vi "ZMQ Rep Test.vi"() -> ()   [LabVIEW 2019, in "RemoteControl.ZMQ.lvlib" / "RemoteControl.ZMQ.lvclass"]
uses:
  RemoteControl.ZMQ.lvclass
  <userlib>/LevyLab/RemoteControl/RemoteControl/Typedefs/Message--Cluster.ctl
  C:/Program Files/National Instruments/LabVIEW 2019/user.lib/LevyLab/RemoteControl/RemoteControl/RemoteControl.lvclass
  <userlib>/LevyLab/RemoteControl/RemoteControl/RemoteControl.lvclass/RemoteControl.ctl
  <vilib>/addons/zeromq/zmq_context.lvclass
  <vilib>/addons/zeromq/socket_type.ctl
  <vilib>/addons/zeromq/zeromq.lvlib
  <vilib>/addons/zeromq/zmq_socket.lvclass
  <vilib>/addons/zeromq/socket_options.ctl
  <userlib>/LevyLab/RemoteControl/RemoteControl/RemoteControl.lvclass
panel:
  out "Message":T1
  out "error out":errorcluster
  in  "stop":bool
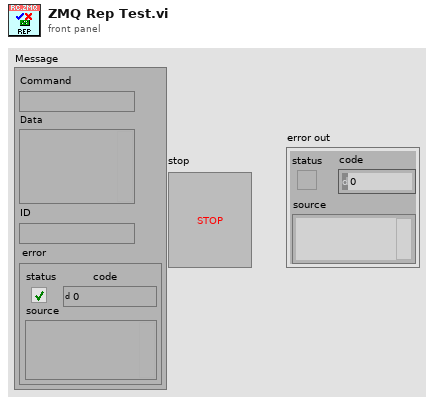
[diagram p1: front panel]
types:
  T1 = typedef "RemoteControl.lvlib/RemoteControl.lvclass/Message--Cluster.ctl" = cluster{"Command":string, "Data":variant, "ID":string, "error":errorcluster}
  T2 = typedef "zeromq.lvlib/socket_options.ctl" = enum8{"NONE", "ZMQ_HWM", "<2>", "ZMQ_SWAP", "ZMQ_AFFINITY", "ZMQ_ROUTING_ID", "ZMQ_SUBSCRIBE", "ZMQ_UNSUBSCRIBE", "ZMQ_RATE", "ZMQ_RECOVERY_IVL", "ZMQ_MCAST_LOOP", "ZMQ_SNDBUF", "ZMQ_RCVBUF", "ZMQ_RCVMORE", "ZMQ_FD", "ZMQ_EVENTS", "ZMQ_TYPE", "ZMQ_LINGER", "ZMQ_RECONNECT_IVL", "ZMQ_BACKLOG", "ZMQ_RECOVERY_IVL_MSEC", "ZMQ_RECONNECT_IVL_MAX", "ZMQ_MAXMSGSIZE", "ZMQ_SNDHWM", "ZMQ_RCVHWM", "ZMQ_MULTICAST_HOPS", "<26>", "ZMQ_RCVTIMEO", "ZMQ_SNDTIMEO", "<29>", "<30>", "ZMQ_IPV4ONLY", "ZMQ_LAST_ENDPOINT", "ZMQ_ROUTER_MANDATORY", "ZMQ_TCP_KEEPALIVE", "ZMQ_TCP_KEEPALIVE_CNT", "ZMQ_TCP_KEEPALIVE_IDLE", "ZMQ_TCP_KEEPALIVE_INTVL", "ZMQ_TCP_ACCEPT_FILTER", "ZMQ_IMMEDIATE", "ZMQ_XPUB_VERBOSE", "ZMQ_ROUTER_RAW", "ZMQ_IPV6", "ZMQ_MECHANISM", "ZMQ_PLAIN_SERVER", "ZMQ_PLAIN_USERNAME", "ZMQ_PLAIN_PASSWORD", "ZMQ_CURVE_SERVER", "ZMQ_CURVE_PUBLICKEY", "ZMQ_CURVE_SECRETKEY", "ZMQ_CURVE_SERVERKEY", "ZMQ_PROBE_ROUTER", "ZMQ_REQ_CORRELATE", "ZMQ_REQ_RELAXED", "ZMQ_CONFLATE", "ZMQ_ZAP_DOMAIN", "ZMQ_ROUTER_HANDOVER", "ZMQ_TOS", "ZMQ_IPC_FILTER_PID", "ZMQ_IPC_FILTER_UID", "ZMQ_IPC_FILTER_GID", "ZMQ_CONNECT_ROUTING_ID", "ZMQ_GSSAPI_SERVER", "ZMQ_GSSAPI_PRINCIPAL", "ZMQ_GSSAPI_SERVICE_PRINCIPAL", "ZMQ_GSSAPI_PLAINTEXT", "ZMQ_HANDSHAKE_IVL", "<67>", "ZMQ_SOCKS_PROXY", "ZMQ_XPUB_NODROP", "ZMQ_BLOCKY", "ZMQ_XPUB_MANUAL", "ZMQ_XPUB_WELCOME_MSG", "ZMQ_STREAM_NOTIFY", "ZMQ_INVERT_MATCHING", "ZMQ_HEARTBEAT_IVL", "ZMQ_HEARTBEAT_TTL", "ZMQ_HEARTBEAT_TIMEOUT", "ZMQ_XPUB_VERBOSER", "ZMQ_CONNECT_TIMEOUT", "ZMQ_TCP_MAXRT", "ZMQ_THREAD_SAFE", "<82>", "<83>", "ZMQ_MULTICAST_MAXTPDU", "ZMQ_VMCI_BUFFER_SIZE", "ZMQ_VMCI_BUFFER_MIN_SIZE", "ZMQ_VMCI_BUFFER_MAX_SIZE", "ZMQ_VMCI_CONNECT_TIMEOUT", "ZMQ_USE_FD", "ZMQ_GSSAPI_PRINCIPAL_NAMETYPE", "ZMQ_GSSAPI_SERVICE_PRINCIPAL_NAMETYPE", "ZMQ_BINDTODEVICE", "ZMQ_ZAP_ENFORCE_DOMAIN", "ZMQ_LOOPBACK_FASTPATH", "ZMQ_METADATA", "ZMQ_MULTICAST_LOOP", "ZMQ_ROUTER_NOTIFY"}
  T3 = typedef "zeromq.lvlib/socket_type.ctl" = enum8{"ZMQ_PAIR", "ZMQ_PUB", "ZMQ_SUB", "ZMQ_REQ", "ZMQ_REP", "ZMQ_DEALER", "ZMQ_ROUTER", "ZMQ_PULL", "ZMQ_PUSH", "ZMQ_XPUB", "ZMQ_XSUB", "ZMQ_STREAM", "ZMQ_SERVER", "ZMQ_CLIENT", "ZMQ_RADIO", "ZMQ_DISH", "ZMQ_GATHER", "ZMQ_SCATTER", "ZMQ_DGRAM"}
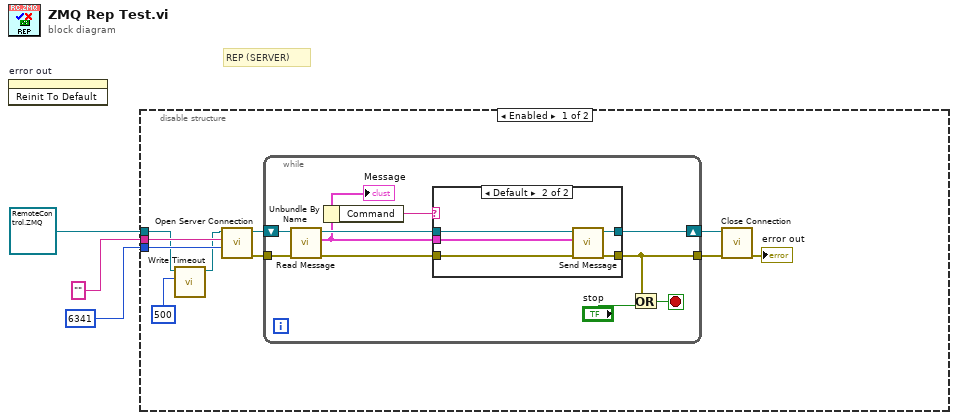
[diagram p0: block diagram]
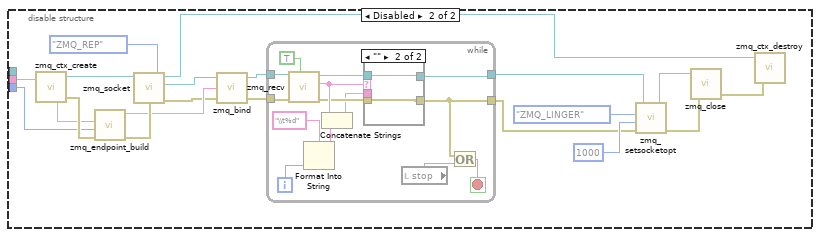
[diagram p3: hidden frame]
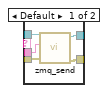
[diagram p4: hidden frame]
diagram:
  # "REP (SERVER)"
  n1 = invoke on="error out" class="Clust (strict)" method="Reinit To Default"() -> ()  [unwired: 3 in, 3 out]
  n2 = disable-structure shown="Enabled" {
    disable-tunnel: refnum<class "RemoteControl.ZMQ.lvclass"> refnum ("RemoteControl.ZMQ.lvlib:RemoteControl.ZMQ.lvclass") -> [w6 _]
    disable-tunnel: u16 6341 ("Port") -> [w9 w38]
    disable-tunnel: "" ("Address") -> [w8 w37]
    frame Enabled {
      n3 = call <userlib>:"Write Timeout.vi"("timeout (ms) [500]"=500 ("timeout in ms (100)"), "RemoteControl in"=w6) -> ("RemoteControl out"=w5:refnum<class "RemoteControl.ZMQ.lvclass">)  [unwired: 8 in, 1 out]
      n4 = call-dynamic "Open Server Connection.vi"("port"=w9, "address"=w8, "RemoteControl.ZMQ in"=w5) -> ("error out"=w12:errorcluster, "RemoteControl.ZMQ out"=w13:refnum<class "RemoteControl.ZMQ.lvclass">)  [unwired: 7 in]
      n5 = while {
        tunnel: w12 -> [w22]
        tunnel: [w18] -> w10
        shift-right: [w19] -> w11
        shift-left: w13 -> [w23]
        stop <- w17 stop-if-true
        n6 = call-dynamic "Read Message.vi"("error in (no error)"=w22, "RemoteControl.ZMQ in"=w23) -> ("error out"=w21:errorcluster, "Message"=w14:T1, "RemoteControl.ZMQ out"=w20:refnum<class "RemoteControl.ZMQ.lvclass">)  [unwired: 7 in]
        "Message" <- w14
        n7 = Unbundle By Name(w14) -> ("Command"=w15:string)
        n8 = case shown="Default" w15 {
          tunnel: w21 -> [w24 w30]
          tunnel: w20 -> [w25 w29]
          tunnel: [w25 w28] -> w19
          tunnel: [w24 w27] -> w18
          tunnel: w14 -> [_ w26]
          frame "" {
            # "no incoming msg:\ndo nothing"
          }
          frame Default {
            n9 = call-dynamic "Send Message.vi"("error in (no error)"=w30, "Message"=w26, "RemoteControl.ZMQ in"=w29) -> ("error out"=w27:errorcluster, "RemoteControl.ZMQ out"=w28:refnum<class "RemoteControl.ZMQ.lvclass">)  [unwired: 7 in]
          }
        }
        n10 = Or(x=w18, y="stop") -> (x .or. y?=w17:bool)
      }
      n11 = call-dynamic "Close Connection.vi"("error in (no error)"=w10, "RemoteControl.ZMQ in"=w11) -> ("error out"=→"error out":errorcluster)  [unwired: 8 in, 1 out]
    }
    frame Disabled {
      n12 = call <vilib>:"zmq_ctx_create.vi"() -> ("error out"=w47:errorcluster, "context out"=w49:refnum<class "zmq_context.lvclass">)  [unwired: 4 in]
      n13 = call <vilib>:"zmq_endpoint_build.vi"("error in"=w47, "port"=w38, "address"=w37) -> ("error out"=w46:errorcluster, "endpoint"=w35:string)  [unwired: 2 in, 1 out]
      n14 = call <vilib>:"zmq_socket.vi"("error in"=w46, "socket type"=socket_type."ZMQ_REP", "context in"=w49) -> ("error out"=w34:errorcluster, "socket out"=w36:refnum<class "zmq_socket.lvclass">, "context out"=w39:refnum<class "zmq_context.lvclass">)  [unwired: 2 in]
      n15 = call <vilib>:"zmq_bind.vi"("error in"=w34, "endpoint"=w35, "socket in"=w36) -> ("error out"=w32:errorcluster, "socket out"=w33:refnum<class "zmq_socket.lvclass">)  [unwired: 1 in]
      n16 = while {
        tunnel: w32 -> [w60]
        tunnel: w33 -> [w61]
        tunnel: [w58] -> w42
        tunnel: [w53] -> w31
        i -> [w56]
        stop <- w62 stop-if-true
        n17 = call <vilib>:"zmq_recv.vi"("no block? (F)"=TRUE, "error in"=w60, "socket in"=w61) -> ("error out"=w51:errorcluster, "data"=w52:string, "socket out"=w59:refnum<class "zmq_socket.lvclass">)  [unwired: 2 in, 2 out]
        n18 = Format Into String(format string="\\t%d" ("Command"), w56) -> (resulting string=w55:string)  [unwired: 2 in, 1 out]
        n19 = Concatenate Strings(w52, w55) -> (w50:string)
        n20 = case shown="\"\"" w52 {
          tunnel: w59 -> [w68 w70]
          tunnel: [w67 w70] -> w58
          tunnel: [w66 w69] -> w53
          tunnel: w51 -> [w64 w69]
          tunnel: w50 -> [w65 _]
          frame Default {
            n21 = call <vilib>:"zmq_send.vi"("error in"=w64, "data"=w65, "socket in"=w68) -> ("error out"=w66:errorcluster, "socket out"=w67:refnum<class "zmq_socket.lvclass">)  [unwired: 4 in]
          }
          frame "" {
          }
        }
        n22 = local read "stop"() -> (w63:bool)
        n23 = Or(x=w53, y=w63) -> (x .or. y?=w62:bool)
      }
      n24 = call <vilib>:"zmq_setsocketopt.vi"("error in"=w31, "value"=1000, "option"=socket_options."ZMQ_LINGER", "socket in"=w42) -> ("error out"=w41:errorcluster, "socket out"=w43:refnum<class "zmq_socket.lvclass">)  [unwired: 2 in]
      n25 = call <vilib>:"zmq_close.vi"("error in"=w41, "socket"=w43) -> ("error out"=w40:errorcluster)  [unwired: 3 in]
      n26 = call <vilib>:"zmq_ctx_destroy.vi"("error in"=w40, "context in"=w39) -> ()  [unwired: 3 in, 1 out]
    }
  }
